vi "_Generate DocMap.vi"(9 "Replace Ref(T)":bool=TRUE, 10 "Array 2":T2[](array[typedef]), 11 "Array":T1[](array[typedef])) -> (3 "Variant":variant)   [LabVIEW 2017, in "csmdoc.lvlib"]
uses:
  csmdoc.lvlib
  _Typedef/DocNote.ctl
  _Typedef/DocElement.ctl
  _Shared/CSM Shared.lvlib
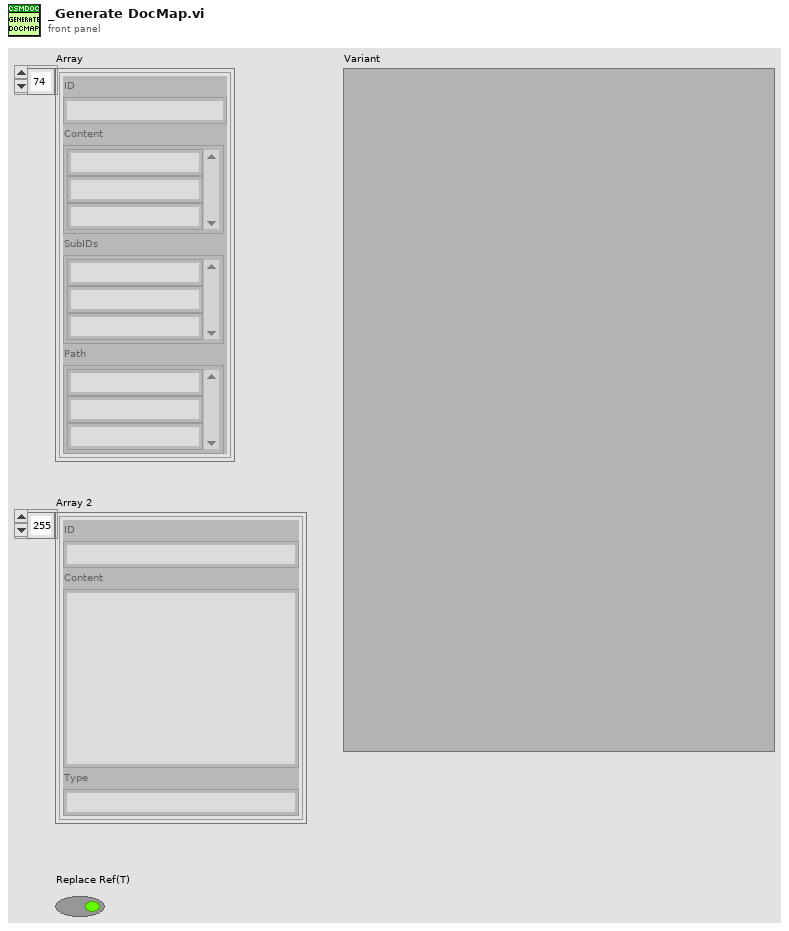
[diagram p1: front panel]
types:
  T1 = typedef "csmdoc.lvlib/DocElement.ctl" = cluster{"ID":string, "Content":string[], "SubIDs":string[], "Path":string[]}
  T2 = typedef "csmdoc.lvlib/DocNote.ctl" = cluster{"ID":string, "Content":string, "Type":string}
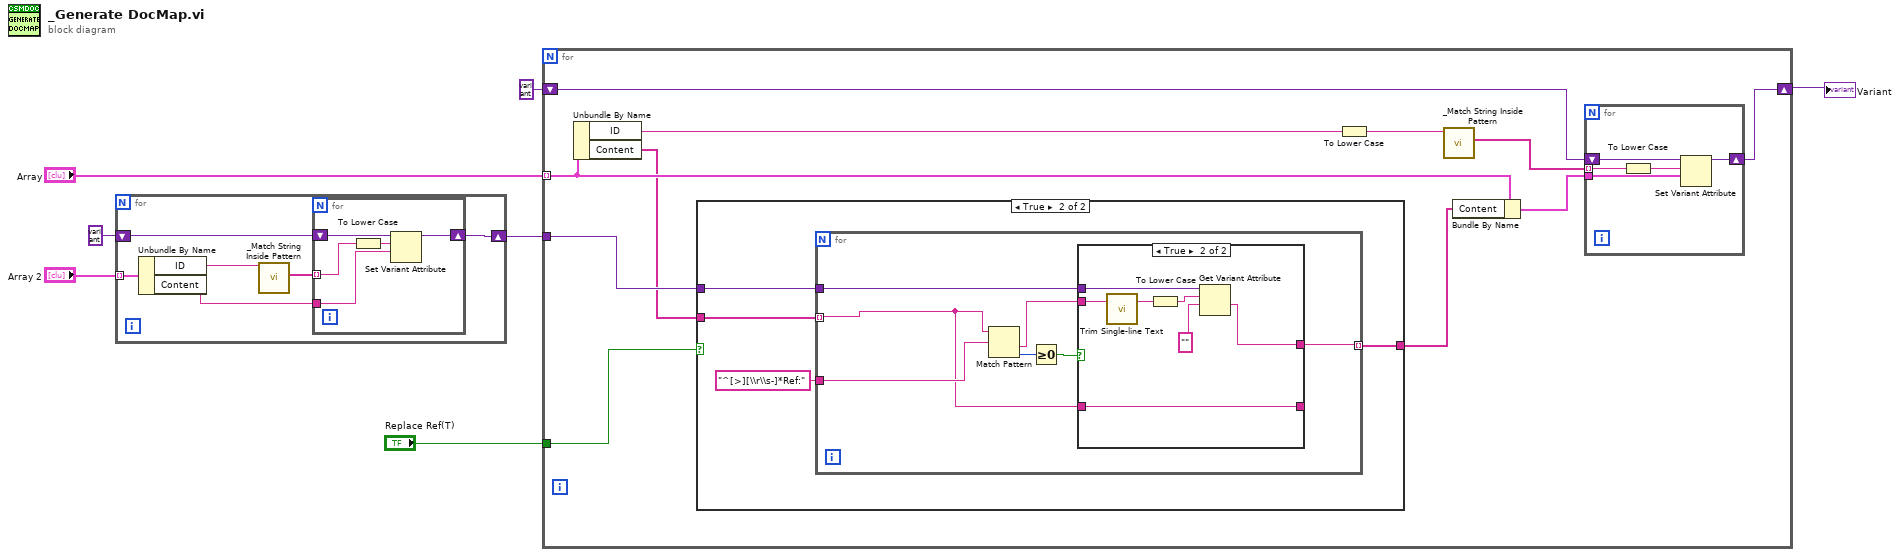
[diagram p0: block diagram]
diagram:
  n1 = for {
    tunnel: "Array 2" -> [w12] mode=indexing
    shift-right: [w9] -> w2
    shift-left: variant -> [w13]
    n2 = Unbundle By Name(w12) -> ("ID"=w11:string, "Content"=w10:string)
    n3 = call "_Match String Inside Pattern.vi"("string"=w11) -> ("Keys"=w8:string[])  [unwired: 9 in, 1 out]
    n4 = for {
      tunnel: w10 -> [w17]
      shift-right: [w16] -> w9
      shift-left: w13 -> [w18]
      tunnel: w8 -> [w15] mode=indexing
      n5 = To Lower Case(string=w15) -> (all lower case string=w14:string)
      n6 = Set Variant Attribute(Variant=w18, name=w14, value=w17) -> (Variant out=w16:variant)  [unwired: 1 in, 2 out]
    }
  }
  n7 = for {
    tunnel: "Array" -> [w24] mode=indexing
    shift-right: [w28] -> w7
    shift-left: variant -> [w29]
    tunnel: w2 -> [w25]
    tunnel: "Replace Ref(T)" -> [w20]
    n8 = Unbundle By Name(w24) -> ("ID"=w27:string, "Content"=w21:string[])
    n9 = case shown="True" w20 {
      tunnel: w25 -> [_ w39]
      tunnel: [w35 w37] -> w23
      tunnel: w21 -> [w35 w36]
      frame False {
      }
      frame True {
        n10 = for {
          tunnel: w36 -> [w40] mode=indexing
          tunnel: w39 -> [w44]
          tunnel: "^[>][\\r\\s-]*Ref:" ("delimited string") -> [w46]
          tunnel: [w41] -> w37 mode=indexing
          n11 = Match Pattern(string=w40, regular expression=w46) -> (after substring=w43:string, offset past match=w45:i32)  [unwired: 1 in, 2 out]
          n12 = Greater Or Equal To 0?(x=w45) -> (x >= 0?=w42:bool)
          n13 = case shown="True" w42 {
            tunnel: w44 -> [_ w54]
            tunnel: w43 -> [_ w52]
            tunnel: [w47 w49] -> w41
            tunnel: w40 -> [w47 w48]
            tunnel: [_ w48] -> _
            frame False {
            }
            frame True {
              n14 = call "Trim Single-line Text.vi"("single-line text"=w52) -> ("trimed text"=w51:string)  [unwired: 2 in]
              n15 = To Lower Case(string=w51) -> (all lower case string=w53:string)
              n16 = Get Variant Attribute(Variant=w54, name=w53, default value (empty Variant)="" ("delimited string")) -> (value=w49:string)  [unwired: 1 in, 3 out]
            }
          }
        }
      }
    }
    n17 = To Lower Case(string=w27) -> (all lower case string=w26:string)
    n18 = call "_Match String Inside Pattern.vi"("string"=w26) -> ("Keys"=w19:string[])  [unwired: 9 in, 1 out]
    n19 = Bundle By Name(cluster=w24, "Content"=w23) -> (w22:T1)
    n20 = for {
      tunnel: w22 -> [w32]
      shift-right: [w33] -> w28
      shift-left: w29 -> [w34]
      tunnel: w19 -> [w31] mode=indexing
      n21 = To Lower Case(string=w31) -> (all lower case string=w30:string)
      n22 = Set Variant Attribute(Variant=w34, name=w30, value=w32) -> (Variant out=w33:variant)  [unwired: 1 in, 2 out]
    }
  }
  "Variant" <- w7
